vi "Experiment Error Policy.vi"(7 "Path":path, 8 "error in (no error)":errorcluster, 10 "error state":string, 11 "Transport in":refnum<class "Transport.lvclass">) -> (0 "handling error":errorcluster, 1 "unhandled error":errorcluster, 2 "COM error?":bool, 3 "message":string)   [LabVIEW 2019, in "Transport.lvclass"]
uses:
  Transport.lvclass
  Transport.lvclass/Transport.ctl
  Control Experiment/Control Experiment.lvclass/Control Experiment.ctl
  <userlib>/_OpenG.lib/error/error.llb/Filter Error Codes (Array)__ogtk.vi
  Control Experiment/Control Experiment.lvclass
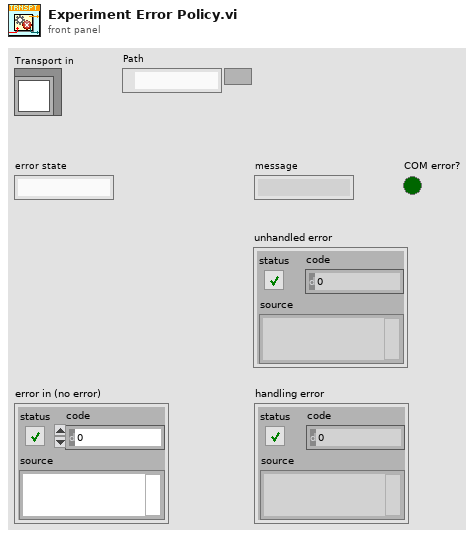
[diagram p1: front panel]
types:
  T1 = enum16{"open", "replace", "create", "open or create", "replace or create", "replace or create with confirmation"}
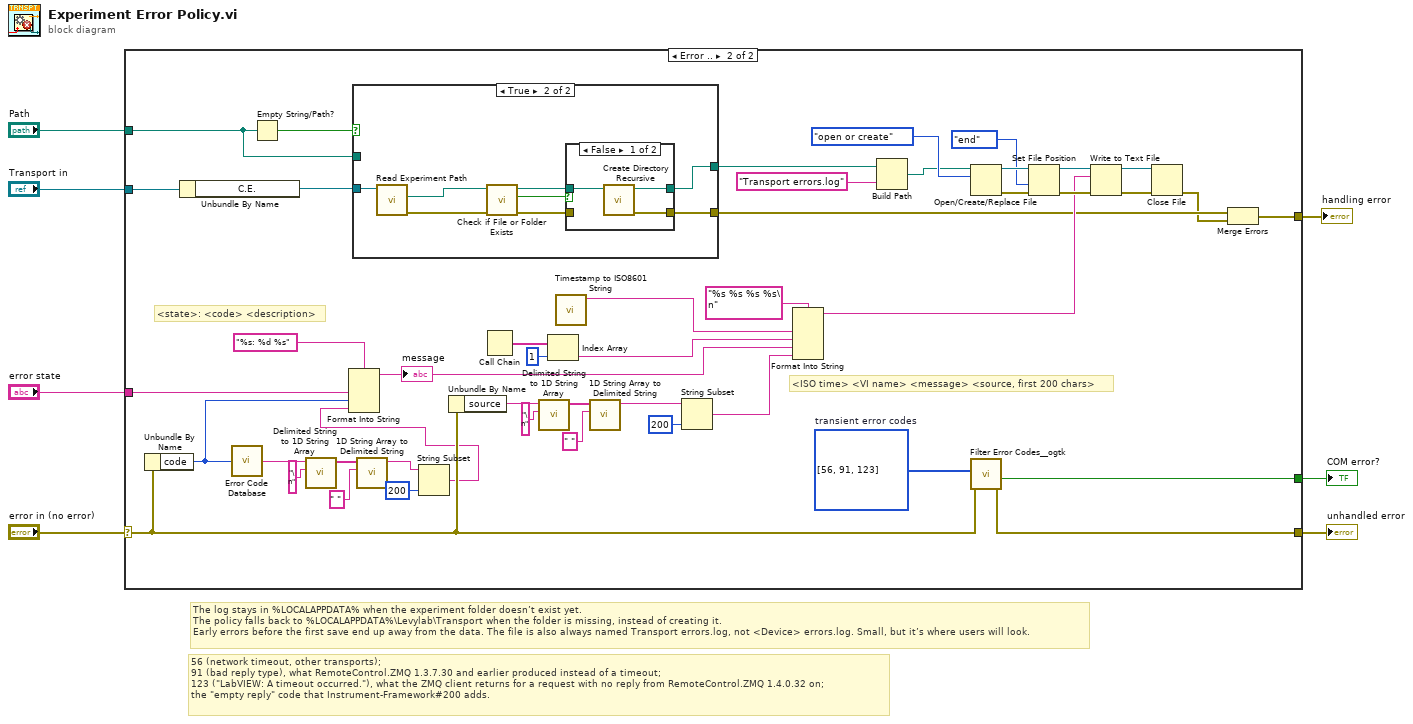
[diagram p0: block diagram]
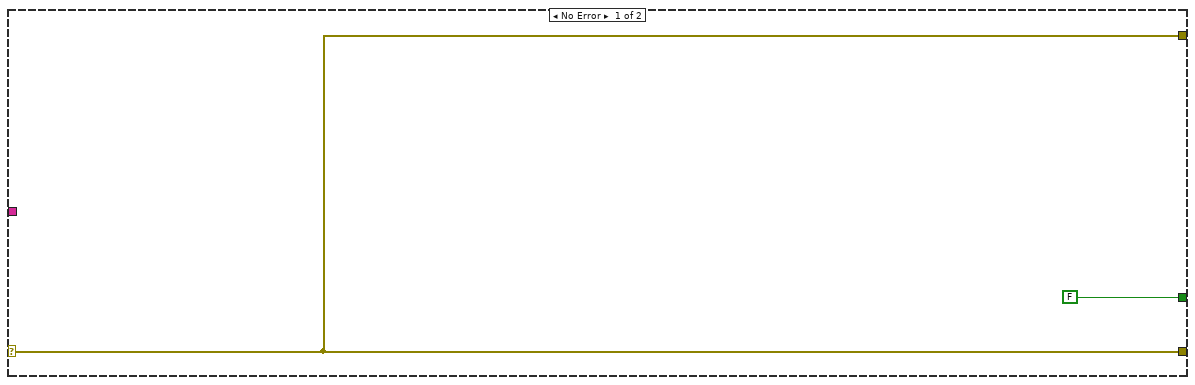
[diagram p2: hidden frame]
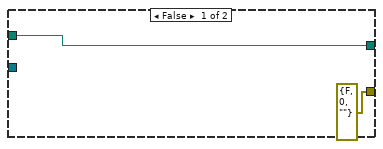
[diagram p3: hidden frame]
diagram:
  # "The log stays in %LOCALAPPDATA% when the experiment folder doesn’t exist yet.\nThe policy falls back to %LOCALAPPDATA%\\Levylab\\Transport when the folder is missing, instead of creating it.\nEarly errors before the first save end up away from the data. The file is also always named Transport errors.log, not <Device> errors.log. Small, but it’s where users will look."
  # "56 (network timeout, other transports);\n91 (bad reply type), what RemoteControl.ZMQ 1.3.7.30 and earlier produced instead of a timeout;\n123 (\"LabVIEW: A timeout occurred.\"), what the ZMQ client returns for a request with no reply from RemoteControl.ZMQ 1.4.0.32 on;\nthe \"empty reply\" code that Instrument-Framework#200 adds."
  n1 = case shown="Error .." "error in (no error)" {
    selector: "error in (no error)" -> [w9 w42]
    tunnel: "Transport in" -> [_ w55]
    tunnel: [FALSE ("Error Filtered?") w53] -> w6
    tunnel: [w9 w52] -> w5
    tunnel: "error state" -> [_ w50]
    tunnel: [w9 w27] -> w2
    tunnel: "Path" -> [_ w23]
    frame No Error {
    }
    frame Error {
      w54 = i32[] [56, 91, 123]  # transient error codes
      # "<ISO time> <VI name> <message> <source, first 200 chars>"
      # "<state>: <code> <description>"
      n2 = Unbundle By Name(w42) -> ("code"=w49:i32)
      n3 = Unbundle By Name(w55) -> ("C.E."=w48:refnum<class "Control Experiment.lvclass">)
      n4 = call <vilib>:"Error Code Database.vi"("Error Code"=w49) -> ("Error Text"=w12:string)
      n5 = Empty String/Path?(string/path=w23) -> (empty?=w24:bool)
      n6 = call <vilib>:"Delimited String to 1D String Array.vi"("delimiter"="\n", "delimited string"=w12) -> ("string array"=w14:string[])  [unwired: 9 in]
      n7 = case shown="True" w24 {
        tunnel: w48 -> [_ w61]
        tunnel: [w57 w62] -> w40
        tunnel: [errorcluster {"status"=FALSE, "code"=0, "source"=""} ("error out") w58] -> w29
        tunnel: w23 -> [w57 _]
        frame False {
        }
        frame True {
          n8 = call "Read Experiment Path.vi"("Control Experiment in"=w61) -> ("error out"=w63:errorcluster, "Experiment Path"=w60:path)  [unwired: 8 in, 1 out]
          n9 = call <vilib>:"Check if File or Folder Exists.vi"("error in (no error)"=w63, "path"=w60) -> ("error out"=w59:errorcluster, "file or folder exists?"=w65:bool, "dup path"=w64:path)  [unwired: 7 in]
          n10 = case shown="False" w65 {
            tunnel: w64 -> [w67 w70]
            tunnel: [w68 w70] -> w62
            tunnel: w59 -> [_ w69]
            tunnel: [w66 w69] -> w58
            frame False {
              n11 = call <vilib>:"Create Directory Recursive.vi"("directory"=w67) -> ("error out"=w66:errorcluster, "directory copy"=w68:path)  [unwired: 4 in, 1 out]
            }
            frame True {
            }
          }
        }
      }
      n12 = call <vilib>:"1D String Array to Delimited String.vi"("delimiter"=" ", "string array"=w14) -> ("delimited string"=w11:string)  [unwired: 9 in]
      n13 = String Subset(string=w11, length (rest)=200 ("length (rest)")) -> (substring=w10:string)  [unwired: 1 in]
      n14 = Format Into String(format string="%s: %d %s", w50, w49, w10) -> (resulting string=w25:string)  [unwired: 2 in, 1 out]
      "message" <- w25
      n15 = Unbundle By Name(w42) -> ("source"=w22:string)
      n16 = Call Chain() -> (call chain=w47:string[])
      n17 = call <vilib>:"Delimited String to 1D String Array.vi"("delimiter"="\n", "delimited string"=w22) -> ("string array"=w20:string[])  [unwired: 9 in]
      n18 = Index Array(array=w47, index=1) -> (element=w43:string)
      n19 = call <vilib>:"Timestamp to ISO8601 String.vi"() -> ("ISO8601 String"=w39:string)  [unwired: 11 in]
      n20 = call <vilib>:"1D String Array to Delimited String.vi"("delimiter"=" ", "string array"=w20) -> ("delimited string"=w18:string)  [unwired: 9 in]
      n21 = String Subset(string=w18, length (rest)=200 ("length (rest)")) -> (substring=w17:string)  [unwired: 1 in]
      n22 = Format Into String(format string="%s %s %s %s\n", w39, w43, w25, w17) -> (resulting string=w30:string)  [unwired: 2 in, 1 out]
      n23 = Build Path(base path=w40, name or relative path="Transport errors.log") -> (appended path=w26:path)
      n24 = Open/Create/Replace File(file path (use dialog)=w26, operation (0:open)=T1."open or create") -> (refnum out=w37:refnum<file>, error out=w35:errorcluster)  [unwired: 4 in, 1 out]
      n25 = call-poly <userlib>:"Filter Error Codes__ogtk.vi"("Error In"=w42, "Error Codes to Filter"=w54) -> ("Error Out"=w52:errorcluster, "Error Filtered?"=w53:bool)  [unwired: 7 in, 1 out]
      n26 = Set File Position(refnum=w37, from (0:start)=enum16{"start", "end", "current"}."end", error in=w35) -> (refnum out=w34:refnum<file>, error out=w31:errorcluster)  [unwired: 1 in]
      n27 = Write to Text File(file (use dialog)=w34, text=w30, error in=w31) -> (refnum out=w33:refnum<file>, error out=w32:errorcluster)  [unwired: 1 in, 1 out]
      n28 = Close File(refnum=w33, error in=w32) -> (error out=w28:errorcluster)  [unwired: 1 out]
      n29 = Merge Errors(w29, w28) -> (w27:errorcluster)
    }
  }
  "unhandled error" <- w5
  "handling error" <- w2
  "COM error?" <- w6
